vi "Teleop.vi"(10 "Match Info":T1={"Autonomous Elapsed Seconds"=0.0, "TeleOp Elapsed Seconds"=0.0, "Disabled Elapsed Seconds"=0.0, "Visited Autonomous"=FALSE, "Visited TeleOp"=FALSE, "Visited Disabled"=FALSE, "Autonomous Settings"={"Autonomous Style"=enum."Independent", "VI Refnum"=refnum}}, 11 "Call Context":T2) -> ()   [LabVIEW 2017]
doc: "This VI is called for each TeleOp packet received from the DS where the robot is not disabled. It is often used to read from the joysticks and update I/O or to update setpoints for timed control loops. It should complete and return within 20 milliseconds or it may miss DS packets."
uses:
  <vilib>/Rock Robotics/WPI/DriverStation/WPI_DriverStationDerivedRobotMode.ctl
  <vilib>/Rock Robotics/WPI/DriverStation/WPI_DriverStationMatch Info.ctl
  PowerUpSrc/Global_Var-RefNum/Joystick_Control.vi
  PowerUpSrc/Global_Var-RefNum/LEDData.vi
  ArgosLib/ArgosLib.lvlib
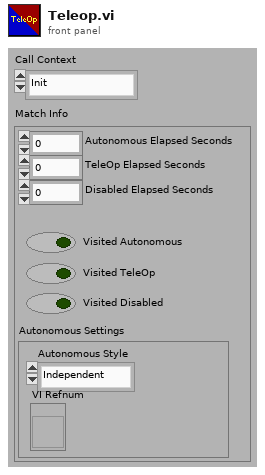
[diagram p1: front panel]
types:
  T1 = typedef "WPI_DriverStationMatch Info.ctl" = cluster{"Autonomous Elapsed Seconds":dbl, "TeleOp Elapsed Seconds":dbl, "Disabled Elapsed Seconds":dbl, "Visited Autonomous":bool, "Visited TeleOp":bool, "Visited Disabled":bool, "Autonomous Settings":cluster{"Autonomous Style":enum16{"Iterative", "Independent"}, "VI Refnum":refnum<vi>}}
  T2 = typedef "WPI_DriverStationDerivedRobotMode.ctl" = enum16{"Init", "Execute", "Stop"}
  T3 = typedef "RobotJoysticks.ctl" = cluster{"Driver Controller":T4, "Operator Controller":T4}
  T4 = typedef "WPI_JoystickDevRef.ctl" = cluster{"Device":T5}
  T5 = typedef "WPI_JoystickDeviceEnum.ctl" = enum16{"USB 0", "USB 1", "USB 2", "USB 3", "USB 4", "USB 5"}
  T6 = typedef "ArgosLib.lvlib/XBoxAxes_Type.ctl" = cluster{"Left_Trigger":dbl, "Right_Trigger ":dbl, "Left_X":dbl, "Left_Y":dbl, "Right_X":dbl, "Right_Y":dbl}
  T7 = typedef "ArgosLib.lvlib/XBoxButtons_Type.ctl" = cluster{"A":bool, "B":bool, "X":bool, " Y":bool, "LB":bool, " RB":bool, "Left_Thumb_Button":bool, "Right_Thumb_Button":bool, "Back":bool, "Start":bool, "Top":bool, "Right":bool, "Bottom":bool, "Left":bool}
  T8 = typedef "JoystickControls.ctl" = cluster{"drive speed":dbl, "drive turning":dbl, "Unassigned_LX":dbl, "Unassigned_RY":dbl, "Cube Release":bool, "Intake Forward":dbl, "Intake Reverse ":dbl, "Switch":bool, "Scale Low":bool, "Scale High":bool, "Shift":bool, "Arm To Preset":bool, "Win_LJ":bool, "Win_RJ":bool, "Swap/ClimbPosition_Back":bool, "Swap_Start":bool, "Arm Extend/Retract":dbl, "Unassigned_RX 2":dbl, "Unassigned_LX 2":dbl, "Arm  Pivot Up/Down ":dbl, "Cube Release 2":bool, "Extend/Retract Intake":dbl, "Open/Close Intake":dbl, "Switch 2":bool, "Scale High 2":bool, "Scale Low 2":bool, "Claw Pinch 2":bool, "Arm Hold":bool, "Unassigned_LJ 2":bool, "Unassigned_RJ 2":bool, "Swap/ClimbPosition_Back 2":bool, "Swap/SelfieStick_Start 2":bool, "Climb Up 2":bool, "Unassigned_Right 2":bool, "Climb Down 2":bool, "Unassigned_Left 2":bool, "Climb Up ":bool, " Unassigned_Right":bool, "Climb Down":bool, "Unassigned_Left":bool}
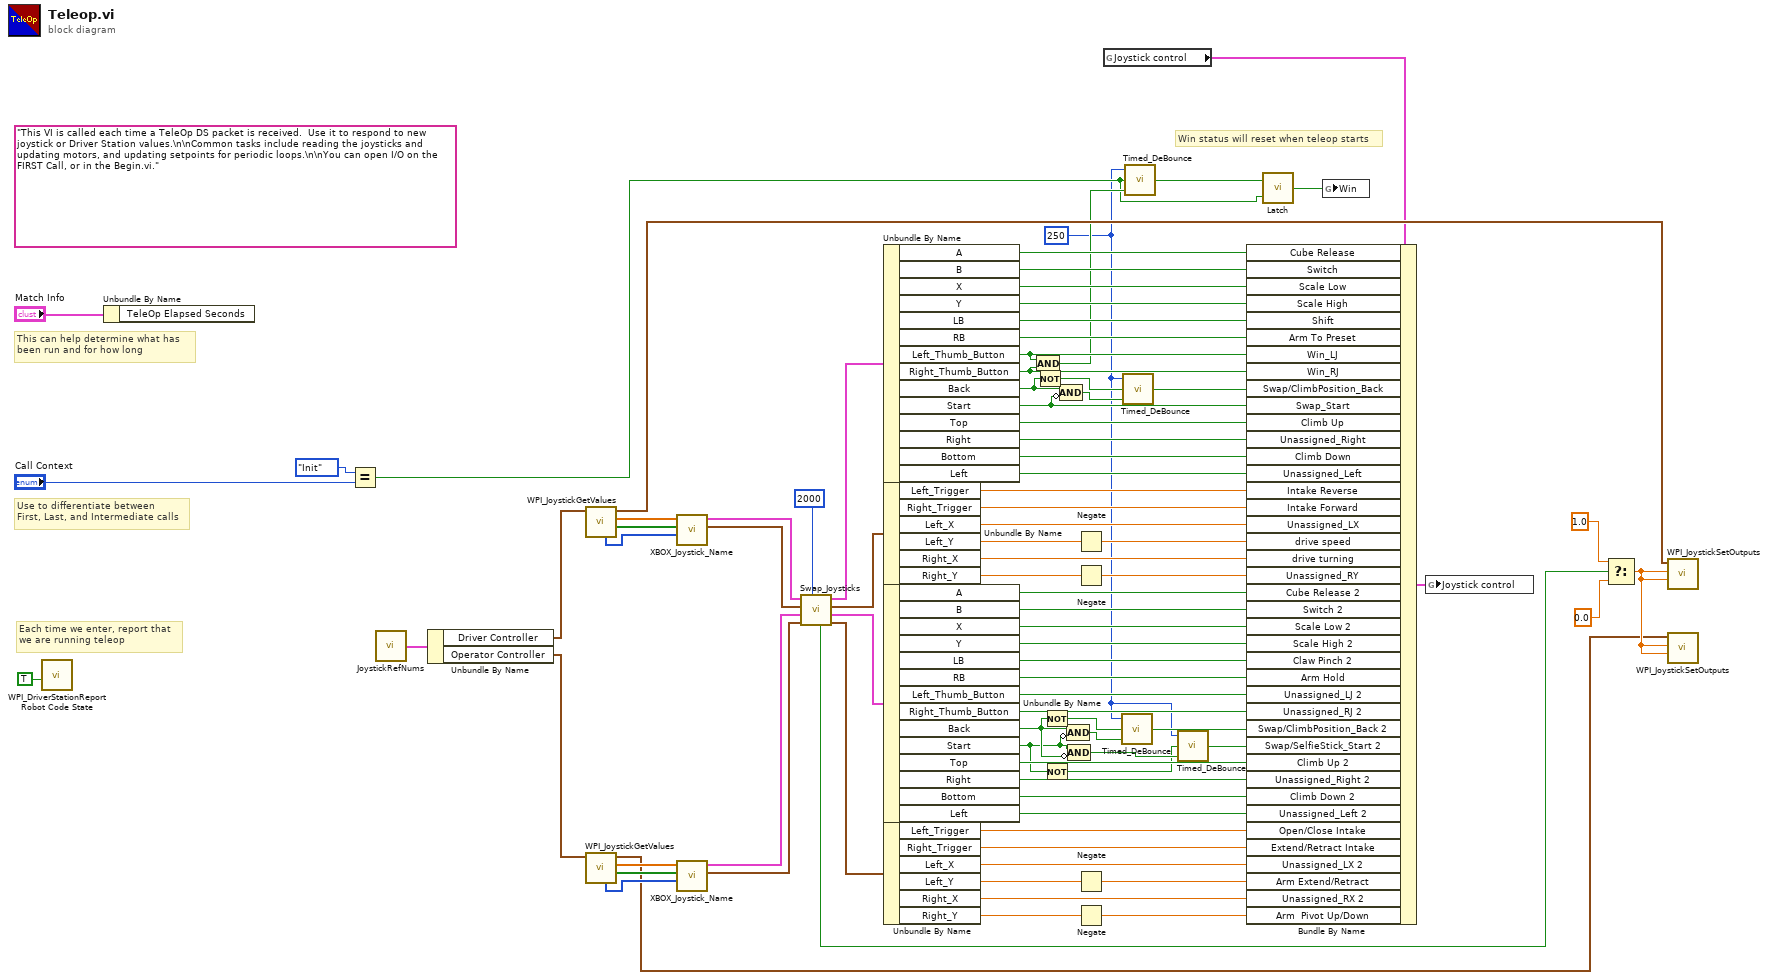
[diagram p0: block diagram]
diagram:
  w5 = u32 250 ("Hold Time(ms)")
  (unwired) "This VI is called each time a TeleOp DS packet is received.  Use it to respond to new joystick or Driver Station values.\n\nCommon tasks include reading the joysticks and updating motors, and updating setpoints for periodic loops.\n\nYou can open I/O on the FIRST Call, or in the Begin.vi."
  # "Win status will reset when teleop starts"
  # "Each time we enter, report that\nwe are running teleop"
  # "Use to differentiate between\nFirst, Last, and Intermediate calls"
  # "This can help determine what has\nbeen run and for how long"
  n1 = call <vilib>:"WPI_DriverStationReport Robot Code State.vi"("TeleOp"=TRUE ("Autonomous")) -> ()  [unwired: 10 in, 1 out]
  n2 = Unbundle By Name("Match Info") -> ()  [unwired: 1 out]
  n3 = Equal?(x=WPI_DriverStationDerivedRobotMode."Init", y="Call Context") -> (x = y?=w10:bool)
  n4 = call "JoystickRefNums.vi"() -> ("Joysticks"=w68:T3)  [unwired: 1 in]
  n5 = Unbundle By Name(w68) -> ("Driver Controller"=w67:T4, "Operator Controller"=w66:T4)
  n6 = call <vilib>:"WPI_JoystickGetValues.vi"("JoystickDevRef"=w67) -> ("Buttons"=w85:bool[], "Axes"=w86:dbl[], "JoystickDevRef"=w77:T4, "POVs"=w65:i16[])  [unwired: 6 in, 1 out]
  n7 = call <vilib>:"WPI_JoystickGetValues.vi"("JoystickDevRef"=w66) -> ("Buttons"=w84:bool[], "Axes"=w83:dbl[], "JoystickDevRef"=w8:T4, "POVs"=w64:i16[])  [unwired: 6 in, 1 out]
  n8 = call "XBOX_Joystick_Name.vi"("POVs"=w65, "Buttons"=w85, "Axes"=w86) -> ("Named Axes"=w73:T6, "Named Buttons"=w74:T7)  [unwired: 7 in]
  n9 = call "XBOX_Joystick_Name.vi"("POVs"=w64, "Buttons"=w84, "Axes"=w83) -> ("Named Axes"=w76:T6, "Named Buttons"=w75:T7)  [unwired: 7 in]
  n10 = call "Swap_Joysticks.vi"("Hold Time(ms)"=u32 2000, "Axes 1 In"=w76, "Buttons 1"=w75, "Axes 0 in"=w73, "Buttons 0"=w74) -> ("Axes 1 out"=w71:T6, "Buttons 1 out"=w70:T7, "Axes 0 out"=w69:T6, "Buttons 0 Out"=w72:T7, "Swap?"=w79:bool)
  n11 = Unbundle By Name(w72) -> ("A"=w62:bool, "B"=w61:bool, "X"=w60:bool, "Y"=w59:bool, "LB"=w58:bool, "RB"=w57:bool, "Left_Thumb_Button"=w17:bool, "Right_Thumb_Button"=w16:bool, "Back"=w23:bool, "Start"=w24:bool, "Top"=w56:bool, "Right"=w55:bool, "Bottom"=w54:bool, "Left"=w53:bool)
  n12 = Unbundle By Name(w69) -> ("Left_Trigger"=w52:dbl, "Right_Trigger"=w51:dbl, "Left_X"=w50:dbl, "Left_Y"=w49:dbl, "Right_X"=w47:dbl, "Right_Y"=w46:dbl)
  n13 = Unbundle By Name(w70) -> ("A"=w44:bool, "B"=w43:bool, "X"=w42:bool, "Y"=w41:bool, "LB"=w40:bool, "RB"=w39:bool, "Left_Thumb_Button"=w38:bool, "Right_Thumb_Button"=w37:bool, "Back"=w3:bool, "Start"=w2:bool, "Top"=w36:bool, "Right"=w35:bool, "Bottom"=w34:bool, "Left"=w33:bool)
  n14 = Unbundle By Name(w71) -> ("Left_Trigger"=w32:dbl, "Right_Trigger"=w31:dbl, "Left_X"=w30:dbl, "Left_Y"=w29:dbl, "Right_X"=w27:dbl, "Right_Y"=w28:dbl)
  n15 = And(x=w17, y=w16) -> (x .and. y?=w15:bool)
  n16 = Not(x=w23) -> (.not. x?=w22:bool)
  n17 = Not(x=w3) -> (.not. x?=w20:bool)
  n18 = Not(x=w2) -> (.not. x?=w1:bool)
  n19 = Compound Arithmetic op=AND(w23, invert w24) -> (w18:bool)
  n20 = Compound Arithmetic op=AND(w3, invert w2) -> (w19:bool)
  n21 = Compound Arithmetic op=AND(w2, invert w3) -> (w4:bool)
  n22 = Negate(x=w49) -> (-x=w48:dbl)
  n23 = Negate(x=w46) -> (-x=w45:dbl)
  n24 = Negate(x=w29) -> (-x=w26:dbl)
  n25 = Negate(x=w28) -> (-x=w25:dbl)
  n26 = global read "Joystick_Control.vi" "Joystick control"() -> (w63:T8)
  n27 = call "Timed_DeBounce.vi"("Input"=w19, "Reset"=w20, "Hold Time(ms)"=w5) -> ("Output"=w7:bool)
  n28 = call "Timed_DeBounce.vi"("Input"=w18, "Reset"=w22, "Hold Time(ms)"=w5) -> ("Output"=w21:bool)
  n29 = call "Timed_DeBounce.vi"("Input"=w15, "Reset"=w10, "Hold Time(ms)"=w5) -> ("Output"=w14:bool)
  n30 = call "Timed_DeBounce.vi"("Input"=w4, "Reset"=w1, "Hold Time(ms)"=w5) -> ("Output"=w6:bool)
  n31 = Bundle By Name(cluster=w63, "Cube Release"=w62, "Switch"=w61, "Scale Low"=w60, "Scale High"=w59, "Shift"=w58, "Arm To Preset"=w57, "Win_LJ"=w17, "Win_RJ"=w16, "Swap/ClimbPosition_Back"=w21, "Swap_Start"=w24, "Climb Up"=w56, "Unassigned_Right"=w55, "Climb Down"=w54, "Unassigned_Left"=w53, "Intake Reverse"=w52, "Intake Forward"=w51, "Unassigned_LX"=w50, "drive speed"=w48, "drive turning"=w47, "Unassigned_RY"=w45, "Cube Release 2"=w44, "Switch 2"=w43, "Scale Low 2"=w42, "Scale High 2"=w41, "Claw Pinch 2"=w40, "Arm Hold"=w39, "Unassigned_LJ 2"=w38, "Unassigned_RJ 2"=w37, "Swap/ClimbPosition_Back 2"=w7, "Swap/SelfieStick_Start 2"=w6, "Climb Up 2"=w36, "Unassigned_Right 2"=w35, "Climb Down 2"=w34, "Unassigned_Left 2"=w33, "Open/Close Intake"=w32, "Extend/Retract Intake"=w31, "Unassigned_LX 2"=w30, "Arm Extend/Retract"=w26, "Unassigned_RX 2"=w27, "Arm  Pivot Up/Down"=w25) -> (w82:T8)
  n32 = call "Latch.vi"("Reset"=w10, "Input"=w14) -> ("LatchOut"=w13:bool)
  n33 = global write "LEDData.vi" "Win"(w13) -> ()
  n34 = global write "Joystick_Control.vi" "Joystick control"(w82) -> ()
  n35 = Select(t=1.0, s=w79, f=0.0) -> (s? t:f=w9:dbl)
  n36 = call <vilib>:"WPI_JoystickSetOutputs.vi"("Right Rumble"=w9, "Left Rumble"=w9, "JoystickDevRef"=w77) -> ()  [unwired: 7 in, 2 out]
  n37 = call <vilib>:"WPI_JoystickSetOutputs.vi"("Right Rumble"=w9, "Left Rumble"=w9, "JoystickDevRef"=w8) -> ()  [unwired: 7 in, 2 out]
